vi "Exp - exec function.vi"(5 "CE InstanceRef":T1, 6 "error in":bool, 9 "ParNum":i32) -> (0 "error out":bool)   [LabVIEW 2021]
doc: "::: CalcExpress Toolkit :::\nCopyright (c) 2000-2026 Konstantin Shifershteyn. All rights reserved."
uses:
  cetypes.llb/CalcExpress Instance RefNum.ctl
  cersrc/celveng32.dll
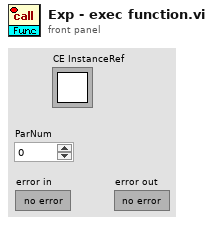
[diagram p1: front panel]
types:
  T1 = typedef "CalcExpress Instance RefNum.ctl" = refnum<k1>
  T2 = cluster{"open to call":bool, "Enable FuncVI2":bool}
  T3 = typedef "CalcExpress Function Argument Info.ctl" = cluster{"type":u32, "str":string, "num":dbl}
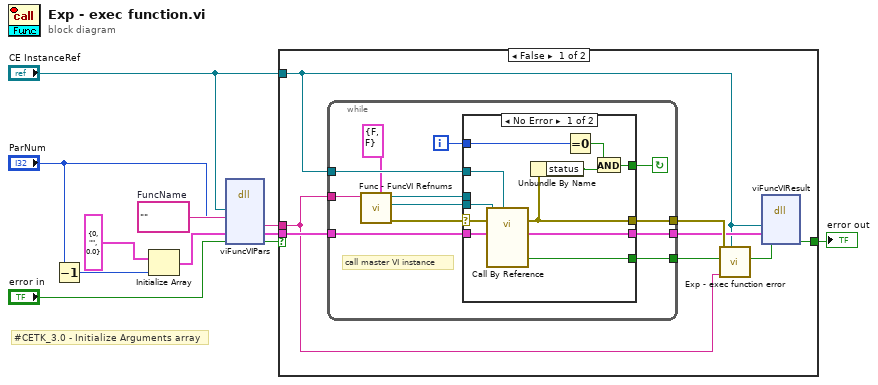
[diagram p0: block diagram]
diagram:
  w9 = ""  # FuncName
  # "#CETK_3.0 - Initialize Arguments array"
  n1 = Decrement(x="ParNum") -> (x-1=w2:i32)
  n2 = Initialize Array(cluster{"type":u32, "str":string, "num":dbl} {"type"=0, "str"="", "num"=0.0} ("expr el out"), w2) -> (w8:cluster{"type":u32, "str":string, "num":dbl}[])
  n3 = dll-call lib="C:/LV Projects/CalcExpress 40 LV2021/vi.lib/addons/CalcExpress/cersrc/celveng*.dll" fn="viFuncVIPars"("iRef"="CE InstanceRef", "nPars"="ParNum", "FuncName"=w9, "ArgList"=w8, "erf"="error in") -> ("FuncName"=w4:string, "ArgList"=w5:cluster{"type":u32, "str":string, "num":dbl}[], "erf"=w6:bool)  [unwired: 6 in, 2 out]
  n4 = case shown="False" w6 {
    selector: w6 -> [_ w44]
    tunnel: [w14 w44] -> w11
    tunnel: "CE InstanceRef" -> [w12 _]
    tunnel: w4 -> [w13 _]
    tunnel: w5 -> [w19 _]
    frame False {
      n5 = while {
        tunnel: [w26] -> w17
        tunnel: w13 -> [w20]
        tunnel: [w28] -> w16
        tunnel: [w27] -> w18
        tunnel: w19 -> [w29]
        tunnel: w12 -> [w24]
        i -> [w31]
        stop <- w30 continue-if-true
        # "call master VI instance"
        n6 = call "Func - FuncVI Refnums.vi"("Params"=T2 {"open to call"=FALSE, "Enable FuncVI2"=FALSE}, "Func name"=w20) -> ("error out"=w23:errorcluster, "FuncVI RefNum out"=w25:refnum<vi>, "FuncVI2 RefNum out"=w22:refnum<vi>)  [unwired: 5 in, 2 out]
        n7 = case shown="No Error" w23 {
          selector: w23 -> [w34 w43]
          tunnel: w31 -> [w42 _]
          tunnel: [w41 _] -> w30
          tunnel: w29 -> [w40 _]
          tunnel: [w39 _] -> w28
          tunnel: [w38 _] -> w27
          tunnel: [w32 w43] -> w26
          tunnel: w25 -> [w33 _]
          tunnel: w24 -> [w35 _]
          tunnel: w22 -> [_ _]
          frame No Error {
            n8 = call-by-ref "Call By Reference"(reference=w33, error in=w34, "InstanceRef"=w35, "arg list"=w40) -> (error out=w32:errorcluster, "error out"=w38:bool, "result"=w39:T3)  [unwired: 6 in, 1 out]
            n9 = Unbundle By Name(w32) -> ("status"=w37:bool)
            n10 = Equal To 0?(x=w42) -> (x = 0?=w36:bool)
            n11 = And(x=w36, y=w37) -> (x .and. y?=w41:bool)
          }
          frame Error {
          }
        }
      }
      n12 = call "Exp - exec function error.vi"("CE InstanceRef"=w12, "func name"=w13, "CE error in"=w18, "error in"=w17) -> ("CE error out"=w15:bool)  [unwired: 5 in]
      n13 = dll-call lib="C:/LV Projects/CalcExpress 40 LV2021/vi.lib/addons/CalcExpress/cersrc/celveng*.dll" fn="viFuncVIResult"("iRef"=w12, "result"=w16, "erf"=w15) -> ("erf"=w14:bool)  [unwired: 6 in, 2 out]
    }
    frame True {
    }
  }
  "error out" <- w11
